vi "ControlRead.vi"(8 "error in":errorcluster, 10 "Selected Properties":string[](array[string]), 11 "Data input":T1) -> (0 "error out":errorcluster, 3 "Data output":T1)   [LabVIEW 2017]
doc: "<B>This VI is used for getting the selelcted property type, value and index, and setting the control value.</B>"
uses:
  Ctrl/Data.ctl
  Ctrl/Caps.ctl
  Ctrl/Property.ctl
  Ctrl/PhysicalChannel.ctl
  Ctrl/Register.ctl
  Ctrl/Bitfield.ctl
  Ctrl/Scale.ctl
  Ctrl/ScaleType.ctl
  Ctrl/Enum.ctl
  Ctrl/EnumValue.ctl
  <vilib>/Utility/miscctls.llb/LVStringsAndValuesArrayTypeDef_U16.ctl
  1b247805-81af-4051-83cb-4bfd180f6ea7.vi
  cd6786a6-1ea5-437c-bd7d-10aa4f833b89.vi
  <vilib>/JDP Science/JSONtext/String Subset.vi
  <vilib>/JDP Science/JSONtext/Parsing/Parse Full Path or Item Name.vi
  <vilib>/JDP Science/JSONtext/Offset/Find Item Locations by Path.vi
  <vilib>/JDP Science/JSONtext/JSON text to Variant.vi
  API/Tree/SLSC Tree Control.lvlib
  <vilib>/JDP Science/JSONtext/JSONtext.lvlib
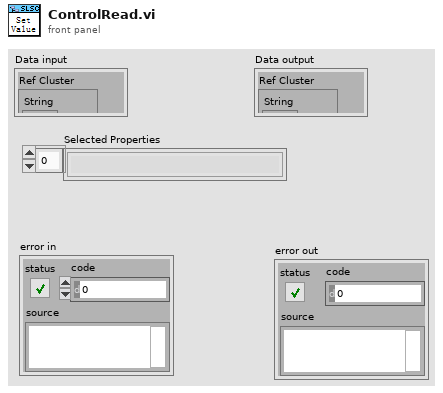
[diagram p1: front panel]
types:
  T1 = typedef "Data.ctl" = cluster{"Ref Cluster":cluster{"String":refnum<vi>, "U8":refnum<vi>, "I8":refnum<vi>, "U32":refnum<vi>, "I32":refnum<vi>, "U64":refnum<vi>, "I64":refnum<vi>, "Ring":refnum<vi>, "DBL":refnum<vi>, "Add":refnum<vi>, "Remove":refnum<vi>, "Property tree":refnum<vi>, "confirm":refnum<vi>}, "JSON Text":string, "Original JSON Text":string, "Caps":T2, "SLSC Output Tree":cluster{"Left Cell String":string, "Child Text":string[], "Child Tag":string, "Item Indent":i32, "Child Only?":bool, "Glyph Index":i32, "offline value":variant}[], "Ref Index and Control Type":cluster{"index":i32, "Datatype":string}, "Selected Type and name":cluster{"Selected Type":enum16{"Property", "Physical Channel", "Other"}, "Selected Property Name":string}, "Update whole Tree?":bool}
  T2 = typedef "Caps.ctl" = cluster{"properties":T3[], "physical channels":T4[], "registers":T5[], "scales":T7[], "enums":T9[], "productName":string}
  T3 = typedef "Property.ctl" = cluster{"name":string, "bitfield":string, "value":variant, "dataType":string, "min":variant, "max":variant, "scale":string, "access":string}
  T4 = typedef "PhysicalChannel.ctl" = cluster{"name":string, "properties":T3[]}
  T5 = typedef "Register.ctl" = cluster{"name":string, "address":i32, "size":i32, "bitfields":T6[], "initialValue":variant, "connectedProperties":string[]}
  T6 = typedef "Bitfield.ctl" = cluster{"name":string, "offset":i32, "size":i32, "signed":bool}
  T7 = typedef "Scale.ctl" = cluster{"name":string, "type":T8, "params":variant}
  T8 = typedef "ScaleType.ctl" = enum16{"NoScale", "Table", "Polynomial", "Linear"}
  T9 = typedef "Enum.ctl" = cluster{"name":string, "values":T10[]}
  T10 = typedef "EnumValue.ctl" = cluster{"name":string, "value":i32}
  T11 = enum16{"Show Selected Control", "All Visiable", "All Invisible"}
  T12 = cluster{"String":refnum<vi>, "U8":refnum<vi>, "I8":refnum<vi>, "U32":refnum<vi>, "I32":refnum<vi>, "U64":refnum<vi>, "I64":refnum<vi>, "Ring":refnum<vi>, "DBL":refnum<vi>, "Add":refnum<vi>, "Remove":refnum<vi>, "Property tree":refnum<vi>, "confirm":refnum<vi>}
  T13 = typedef "LVStringsAndValuesArrayTypeDef_U16.ctl" = cluster{"String":string, "Value":u16}[]
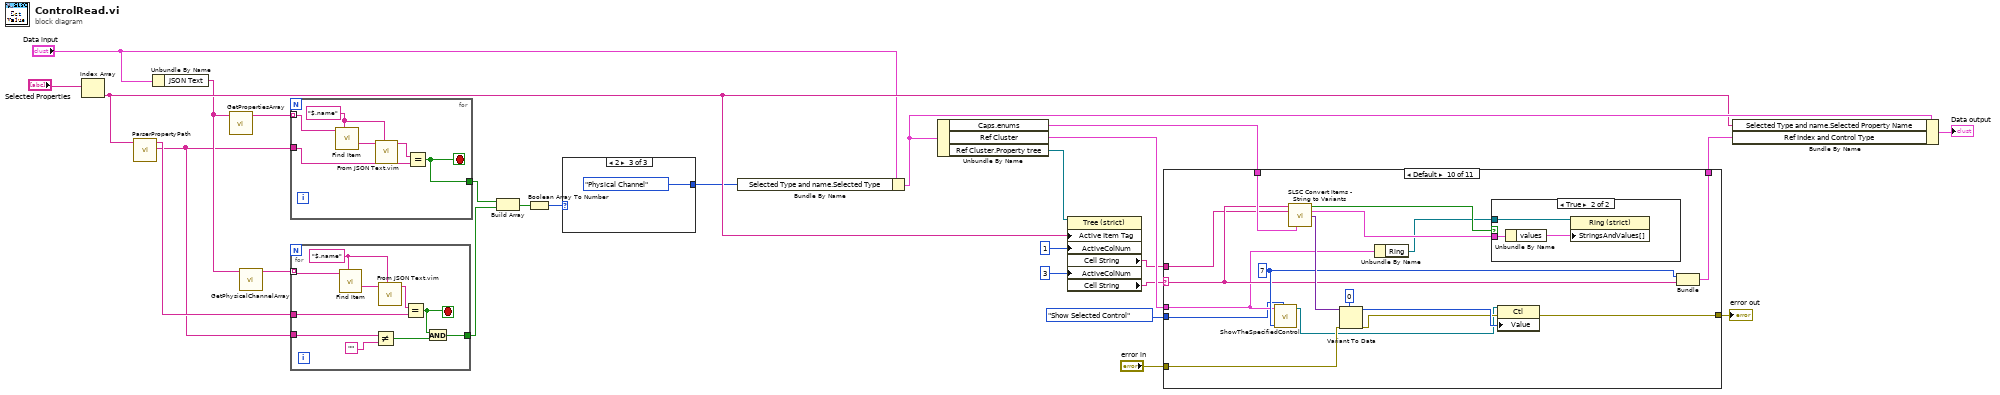
[diagram p0: block diagram]
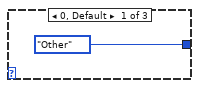
[diagram p2: hidden frame]
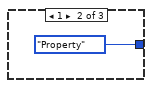
[diagram p3: hidden frame]
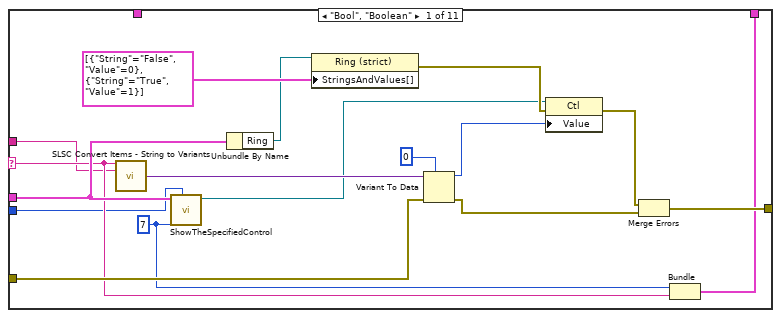
[diagram p4: hidden frame]
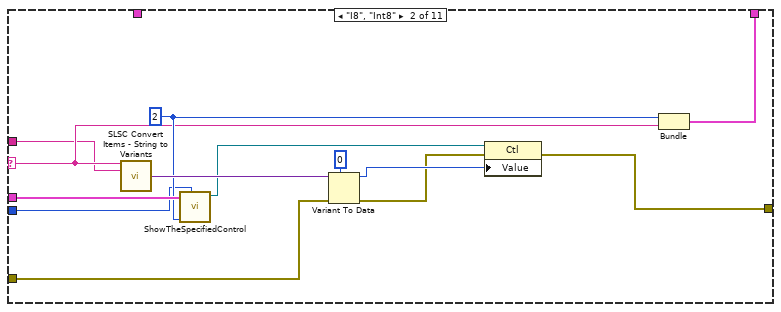
[diagram p5: hidden frame]
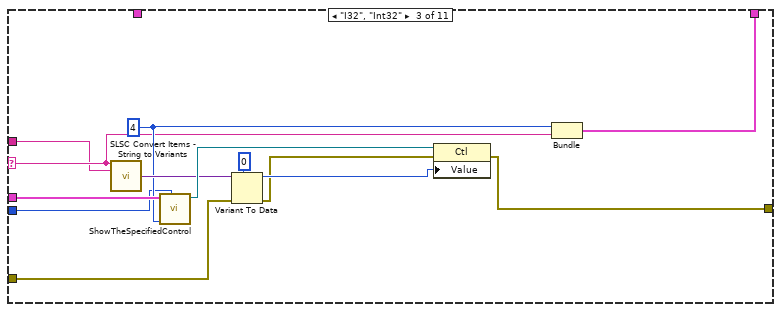
[diagram p6: hidden frame]
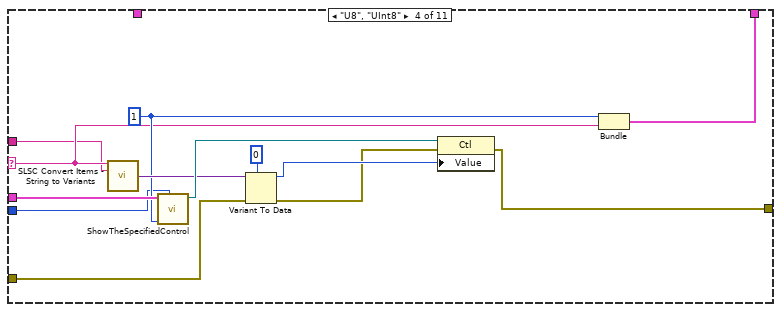
[diagram p7: hidden frame]
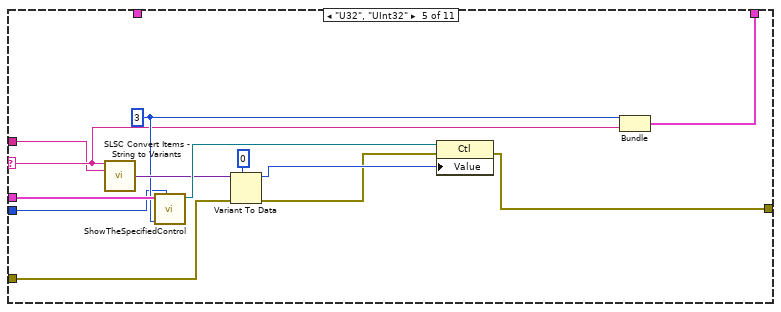
[diagram p8: hidden frame]
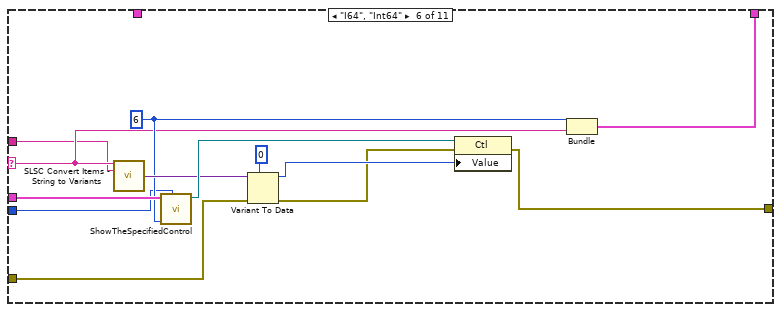
[diagram p9: hidden frame]
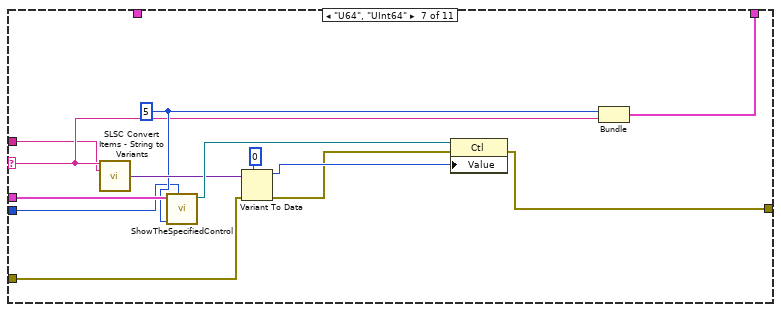
[diagram p10: hidden frame]
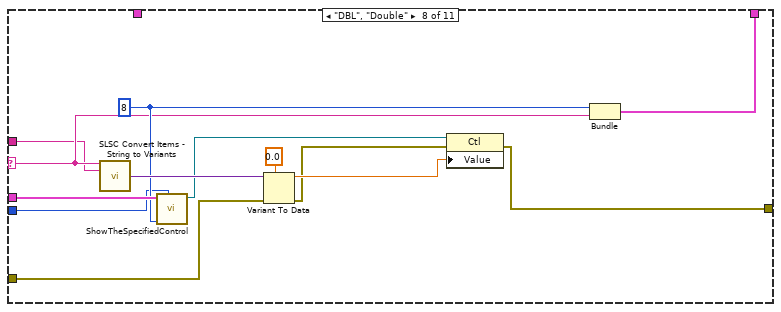
[diagram p11: hidden frame]
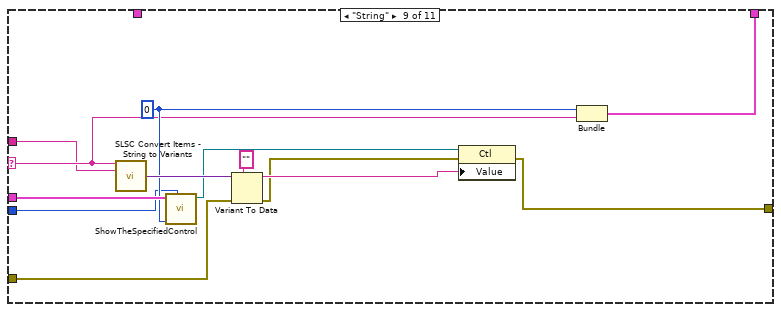
[diagram p12: hidden frame]
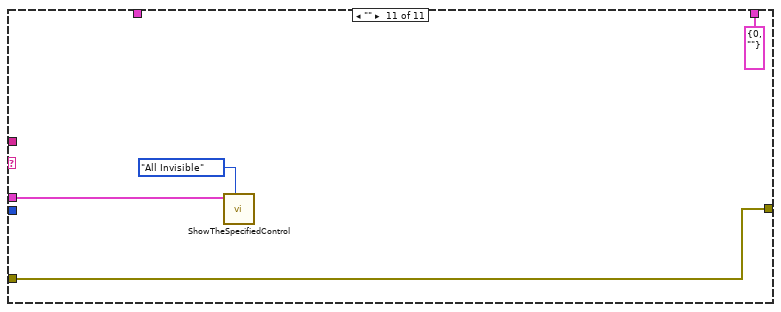
[diagram p14: hidden frame]
diagram:
  n1 = Index Array(array="Selected Properties") -> (element=w13:string)  [unwired: 1 in]
  n2 = call "ParserPropertyPath.vi"("Seleted Item Name"=w13) -> ("Property"=w1:string, "Physical channel"=w9:string)  [unwired: 7 in]
  n3 = Unbundle By Name("Data input") -> ("JSON Text"=w11:string)
  n4 = call "GetPropertiesArray.vi"("JSON Text"=w11) -> ("Properties Array"=w12:string[])  [unwired: 9 in, 1 out]
  n5 = call "GetPhysicalChannelArray.vi"("JSON Text"=w11) -> ("PhysicalChannels Array"=w10:string[])  [unwired: 9 in, 1 out]
  n6 = for {
    tunnel: w12 -> [w32] mode=indexing
    tunnel: w1 -> [w27]
    tunnel: [w28] -> w8
    stop <- w28 stop-if-true
    w30 = "$.name" ("$Path or Item Name")
    n7 = call <vilib>:"Find Item.vi"("$Path or Item Name"=w30, "JSON"=w32) -> ("<JSON>"=w31:string)  [unwired: 6 in, 3 out]
    n8 = call "From JSON Text.vim"("Data Type and Default Value"=w30, "JSON"=w31) -> ("Data out"=w29:string)  [unwired: 8 in, 1 out]
    n9 = Equal?(x=w29, y=w27) -> (x = y?=w28:bool)
  }
  n10 = for {
    tunnel: w10 -> [w42] mode=indexing
    tunnel: w9 -> [w38]
    tunnel: [w36] -> w7
    tunnel: w1 -> [w35]
    stop <- w37 stop-if-true
    w40 = "$.name" ("$Path or Item Name")
    n11 = call <vilib>:"Find Item.vi"("$Path or Item Name"=w40, "JSON"=w42) -> ("<JSON>"=w41:string)  [unwired: 6 in, 3 out]
    n12 = Not Equal?(x=w35, y="") -> (x != y?=w33:bool)
    n13 = call "From JSON Text.vim"("Data Type and Default Value"=w40, "JSON"=w41) -> ("Data out"=w39:string)  [unwired: 8 in, 1 out]
    n14 = Equal?(x=w39, y=w38) -> (x = y?=w37:bool)
    n15 = And(x=w37, y=w33) -> (x .and. y?=w36:bool)
  }
  n16 = Build Array(w8, w7) -> (w6:bool[])
  n17 = Boolean Array To Number(Boolean array=w6) -> (number=w5:u32)
  n18 = case shown="2" w5 {
    tunnel: [enum16{"Property", "Physical Channel", "Other"}."Other" ("Selected Type and name.Selected Type") enum16{"Property", "Physical Channel", "Other"}."Property" ("Selected Type and name.Selected Type") enum16{"Property", "Physical Channel", "Other"}."Physical Channel" ("Selected Type and name.Selected Type")] -> w4
    frame 0, Default {
    }
    frame 1 {
    }
    frame 2 {
    }
  }
  n19 = Bundle By Name(cluster="Data input", "Selected Type and name.Selected Type"=w4) -> (w21:T1)
  n20 = Unbundle By Name(w21) -> ("Caps.enums"=w26:T9[], "Ref Cluster"=w25:T12, "Ref Cluster.Property tree"=w18:refnum<vi>)
  n21 = property class="Tree (strict)"(reference=w18, "Active Item Tag"=w13, "ActiveColNum"=1 ("Active Cell:Active Column Number"), "ActiveColNum"=3 ("Active Cell:Active Column Number")) -> ("Cell String"=w15:string, "Cell String"=w14:string)  [unwired: 1 in, 2 out]
  n22 = case shown="Default" w14 {
    selector: w14 -> [w49 w66 w79 w92 w105 w118 w131 w144 w157 w172 _]
    tunnel: [w55 w70 w81 w94 w107 w120 w133 w146 w159 w175 w188] -> w22
    tunnel: "error in" -> [w56 w68 w83 w96 w109 w122 w135 w148 w161 w177 w188]
    tunnel: w26 -> [_ _ _ _ _ _ _ _ _ w178 _]
    tunnel: w25 -> [w52 w71 w84 w97 w110 w123 w136 w149 w162 w170 w187]
    tunnel: [w48 w65 w78 w91 w104 w117 w130 w143 w156 w171 cluster{"index":i32, string} {"index"=0, ""}] -> w23
    tunnel: w15 -> [w47 w64 w77 w90 w103 w116 w129 w142 w155 w168 _]
    tunnel: T11."Show Selected Control" ("Command") -> [w46 w63 w76 w89 w102 w115 w128 w141 w154 w167 _]
    frame "Bool", "Boolean" {
      w50 = 7 ("index")
      n23 = call "SLSC Convert Items - String to Variants.vi"("Datatype"=w49, "Value"=w47) -> ("Value"=w61:variant)  [unwired: 11 in, 2 out]
      n24 = call "ShowTheSpecifiedControl.vi"("Command"=w46, "index"=w50, "Ref Cluster"=w52) -> ("element"=w57:refnum<vi>)  [unwired: 8 in]
      n25 = Unbundle By Name(w52) -> ("Ring"=w51:refnum<vi>)
      n26 = property on="Property Node" class="Ring (strict)"(reference=w51, "StringsAndValues[]"=T13 [{"String"="False", "Value"=0}, {"String"="True", "Value"=1}] ("Strings And Values []")) -> (error out=w58:errorcluster)  [unwired: 1 in, 1 out]
      n27 = Variant To Data(error in=w56, type=u16 0 ("Value"), Variant=w61) -> (data=w60:u16, error out=w53:errorcluster)
      n28 = property class="Ctl"(reference=w57, error in=w58, "Value"=w60) -> (error out=w54:errorcluster)  [unwired: 1 out]
      n29 = Merge Errors(w54, w53) -> (w55:errorcluster)
      n30 = Bundle("index"=w50, w49) -> (w48:cluster{"index":i32, string})  [unwired: 1 in]
    }
    frame "I8", "Int8" {
      w67 = 2 ("index")
      n31 = call "SLSC Convert Items - String to Variants.vi"("Datatype"=w66, "Value"=w64) -> ("Value"=w74:variant)  [unwired: 11 in, 2 out]
      n32 = call "ShowTheSpecifiedControl.vi"("Command"=w63, "index"=w67, "Ref Cluster"=w71) -> ("element"=w72:refnum<vi>)  [unwired: 8 in]
      n33 = Variant To Data(error in=w68, type=i8 0 ("Value"), Variant=w74) -> (data=w73:i8, error out=w69:errorcluster)
      n34 = property class="Ctl"(reference=w72, error in=w69, "Value"=w73) -> (error out=w70:errorcluster)  [unwired: 1 out]
      n35 = Bundle("index"=w67, w66) -> (w65:cluster{"index":i32, string})  [unwired: 1 in]
    }
    frame "I32", "Int32" {
      w80 = 4 ("index")
      n36 = call "SLSC Convert Items - String to Variants.vi"("Datatype"=w79, "Value"=w77) -> ("Value"=w85:variant)  [unwired: 11 in, 2 out]
      n37 = call "ShowTheSpecifiedControl.vi"("Command"=w76, "index"=w80, "Ref Cluster"=w84) -> ("element"=w87:refnum<vi>)  [unwired: 8 in]
      n38 = Variant To Data(error in=w83, type=0 ("Value"), Variant=w85) -> (data=w86:i32, error out=w82:errorcluster)
      n39 = property class="Ctl"(reference=w87, error in=w82, "Value"=w86) -> (error out=w81:errorcluster)  [unwired: 1 out]
      n40 = Bundle("index"=w80, w79) -> (w78:cluster{"index":i32, string})  [unwired: 1 in]
    }
    frame "U8", "UInt8" {
      w93 = 1 ("index")
      n41 = call "SLSC Convert Items - String to Variants.vi"("Datatype"=w92, "Value"=w90) -> ("Value"=w98:variant)  [unwired: 11 in, 2 out]
      n42 = call "ShowTheSpecifiedControl.vi"("Command"=w89, "index"=w93, "Ref Cluster"=w97) -> ("element"=w100:refnum<vi>)  [unwired: 8 in]
      n43 = Variant To Data(error in=w96, type=u8 0 ("Value"), Variant=w98) -> (data=w99:u8, error out=w95:errorcluster)
      n44 = property class="Ctl"(reference=w100, error in=w95, "Value"=w99) -> (error out=w94:errorcluster)  [unwired: 1 out]
      n45 = Bundle("index"=w93, w92) -> (w91:cluster{"index":i32, string})  [unwired: 1 in]
    }
    frame "U32", "UInt32" {
      w106 = 3 ("index")
      n46 = call "SLSC Convert Items - String to Variants.vi"("Datatype"=w105, "Value"=w103) -> ("Value"=w111:variant)  [unwired: 11 in, 2 out]
      n47 = call "ShowTheSpecifiedControl.vi"("Command"=w102, "index"=w106, "Ref Cluster"=w110) -> ("element"=w113:refnum<vi>)  [unwired: 8 in]
      n48 = Variant To Data(error in=w109, type=u32 0 ("Value"), Variant=w111) -> (data=w112:u32, error out=w108:errorcluster)
      n49 = property class="Ctl"(reference=w113, error in=w108, "Value"=w112) -> (error out=w107:errorcluster)  [unwired: 1 out]
      n50 = Bundle("index"=w106, w105) -> (w104:cluster{"index":i32, string})  [unwired: 1 in]
    }
    frame "I64", "Int64" {
      w119 = 6 ("index")
      n51 = call "SLSC Convert Items - String to Variants.vi"("Datatype"=w118, "Value"=w116) -> ("Value"=w124:variant)  [unwired: 11 in, 2 out]
      n52 = call "ShowTheSpecifiedControl.vi"("Command"=w115, "index"=w119, "Ref Cluster"=w123) -> ("element"=w126:refnum<vi>)  [unwired: 8 in]
      n53 = Variant To Data(error in=w122, type=i64 0 ("Value"), Variant=w124) -> (data=w125:i64, error out=w121:errorcluster)
      n54 = property class="Ctl"(reference=w126, error in=w121, "Value"=w125) -> (error out=w120:errorcluster)  [unwired: 1 out]
      n55 = Bundle("index"=w119, w118) -> (w117:cluster{"index":i32, string})  [unwired: 1 in]
    }
    frame "U64", "UInt64" {
      w132 = 5 ("index")
      n56 = call "SLSC Convert Items - String to Variants.vi"("Datatype"=w131, "Value"=w129) -> ("Value"=w137:variant)  [unwired: 11 in, 2 out]
      n57 = call "ShowTheSpecifiedControl.vi"("Command"=w128, "index"=w132, "Ref Cluster"=w136) -> ("element"=w139:refnum<vi>)  [unwired: 8 in]
      n58 = Variant To Data(error in=w135, type=u64 0, Variant=w137) -> (data=w138:u64, error out=w134:errorcluster)
      n59 = property class="Ctl"(reference=w139, error in=w134, "Value"=w138) -> (error out=w133:errorcluster)  [unwired: 1 out]
      n60 = Bundle("index"=w132, w131) -> (w130:cluster{"index":i32, string})  [unwired: 1 in]
    }
    frame "DBL", "Double" {
      w145 = 8 ("index")
      n61 = call "SLSC Convert Items - String to Variants.vi"("Datatype"=w144, "Value"=w142) -> ("Value"=w151:variant)  [unwired: 11 in, 2 out]
      n62 = call "ShowTheSpecifiedControl.vi"("Command"=w141, "index"=w145, "Ref Cluster"=w149) -> ("element"=w150:refnum<vi>)  [unwired: 8 in]
      n63 = Variant To Data(error in=w148, type=0.0 ("Value"), Variant=w151) -> (data=w152:dbl, error out=w147:errorcluster)
      n64 = property class="Ctl"(reference=w150, error in=w147, "Value"=w152) -> (error out=w146:errorcluster)  [unwired: 1 out]
      n65 = Bundle("index"=w145, w144) -> (w143:cluster{"index":i32, string})  [unwired: 1 in]
    }
    frame "String" {
      w158 = 0 ("index")
      n66 = call "SLSC Convert Items - String to Variants.vi"("Datatype"=w157, "Value"=w155) -> ("Value"=w164:variant)  [unwired: 11 in, 2 out]
      n67 = call "ShowTheSpecifiedControl.vi"("Command"=w154, "index"=w158, "Ref Cluster"=w162) -> ("element"=w163:refnum<vi>)  [unwired: 8 in]
      n68 = Variant To Data(error in=w161, type="" ("Value"), Variant=w164) -> (data=w165:string, error out=w160:errorcluster)
      n69 = property class="Ctl"(reference=w163, error in=w160, "Value"=w165) -> (error out=w159:errorcluster)  [unwired: 1 out]
      n70 = Bundle("index"=w158, w157) -> (w156:cluster{"index":i32, string})  [unwired: 1 in]
    }
    frame Default {
      w173 = 7 ("index")
      n71 = call "ShowTheSpecifiedControl.vi"("Command"=w167, "index"=w173, "Ref Cluster"=w170) -> ("element"=w174:refnum<vi>)  [unwired: 8 in]
      n72 = call "SLSC Convert Items - String to Variants.vi"("Datatype"=w172, "Value"=w168, "enums"=w178) -> ("Datatype found?"=w179:bool, "enum"=w180:T9, "Value"=w182:variant)  [unwired: 10 in]
      n73 = Variant To Data(error in=w177, type=0 ("Value"), Variant=w182) -> (data=w181:i32, error out=w176:errorcluster)
      n74 = Unbundle By Name(w170) -> ("Ring"=w169:refnum<vi>)
      n75 = case shown="True" w179 {
        tunnel: w180 -> [_ w186]
        tunnel: w169 -> [_ w184]
        frame False {
        }
        frame True {
          n76 = Unbundle By Name(w186) -> ("values"=w185:T10[])
          n77 = property on="Property Node" class="Ring (strict)"(reference=w184, "StringsAndValues[]"=w185) -> ()  [unwired: 1 in, 2 out]
        }
      }
      n78 = property class="Ctl"(reference=w174, error in=w176, "Value"=w181) -> (error out=w175:errorcluster)  [unwired: 1 out]
      n79 = Bundle("index"=w173, w172) -> (w171:cluster{"index":i32, string})  [unwired: 1 in]
    }
    frame "" {
      n80 = call "ShowTheSpecifiedControl.vi"("Command"=T11."All Invisible", "Ref Cluster"=w187) -> ()  [unwired: 9 in, 1 out]
    }
  }
  "error out" <- w22
  n81 = Bundle By Name(cluster=w21, "Selected Type and name.Selected Property Name"=w13, "Ref Index and Control Type"=w23) -> (→"Data output":T1)
